vi "Supervisor_Finalize_Run.vi"(8 "error in (no error)":errorcluster={"status"=FALSE, "code"=0, "source"="\"\""}, 10 "results and events":string, 11 "RunContext":string) -> (0 "error out":errorcluster={"status"=FALSE, "code"=0, "source"="\"\""}, 2 "status ok":bool, 3 "Final run status":string)   [LabVIEW 2026]
doc: "INTENT: Finalize run after control secured. LOGIC: Mark incomplete operations, commit run outcome, close capture sessions and release resources."
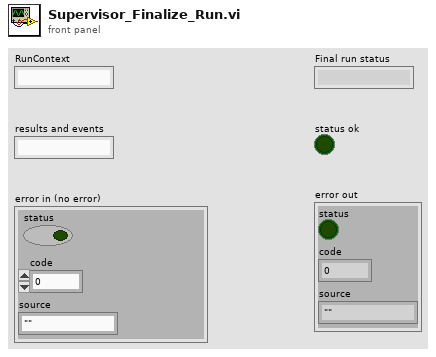
[diagram p1: front panel]
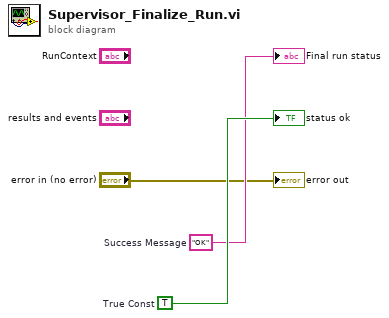
[diagram p0: block diagram]
diagram:
  w3 = TRUE  # True Const
  w2 = "OK"  # Success Message
  "Final run status" <- w2
  "status ok" <- w3
  "error out" <- "error in (no error)"
